vi "Progress Window.vi"(9 "Stop":refnum<data-value>, 10 "Progress":refnum<data-value>, 11 "Status String":refnum<data-value>) -> ()   [LabVIEW 2017, in "Build Automation.lvlib"]
uses:
  Build Automation.lvlib
panel:
  out "Status Message":string
  out "Progress":dbl(slide) scale=0.0..1.0 scale format="%.1f"
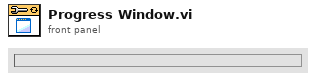
[diagram p1: front panel]
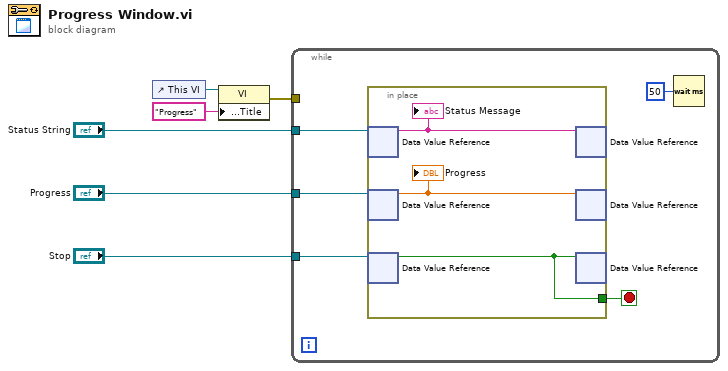
[diagram p0: block diagram]
diagram:
  n1 = control-ref of="This VI"() -> (w3:refnum<vi>)
  n2 = property class="VI"(reference=w3, "Front Panel.Title"="Progress" ("Front Panel Window:Title")) -> (error out=w2:errorcluster)  [unwired: 1 in, 1 out]
  n3 = while {
    tunnel: "Status String" -> [w10]
    tunnel: "Stop" -> [w9]
    tunnel: "Progress" -> [w7]
    tunnel: w2 -> [_]
    stop <- w8 stop-if-true
    n4 = in-place {
      in-place-border: [w13] -> w8
      n5 = in-place-dvr #1(w10) -> (w14:string)  [unwired: 1 out]
      "Status Message" <- w14
      n6 = in-place-dvr #2(w7) -> (w12:dbl)  [unwired: 1 out]
      "Progress" <- w12
      n7 = in-place-dvr #3(w9) -> (w13:bool)  [unwired: 1 out]
      n8 = in-place-dvr #1(w14) -> ()  [unwired: 2 out]
      n9 = in-place-dvr #2(w12) -> ()  [unwired: 2 out]
      n10 = in-place-dvr #3(w13) -> ()  [unwired: 2 out]
    }
    n11 = Wait (ms)(milliseconds to wait=u32 50) -> ()  [unwired: 1 out]
  }
